vi "lvmcp_ctltype.vi"() -> ()   [LabVIEW 2026]
panel:
  out "error out":errorcluster
  out "data bytes":u8[](array[numeric])
  out "type string":i16[](array[numeric])
  in  "reference":refnum<vi>
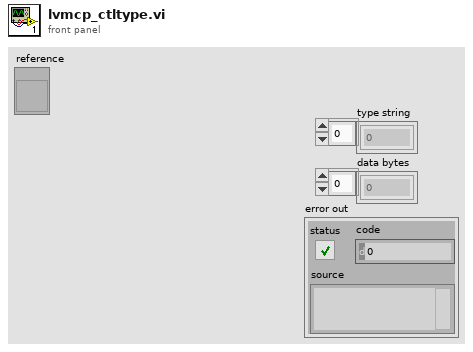
[diagram p1: front panel]
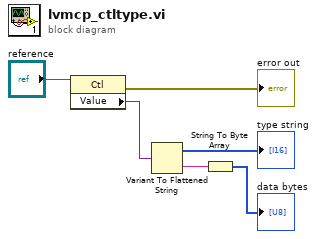
[diagram p0: block diagram]
diagram:
  n1 = property class="Ctl"(reference="reference") -> (error out=→"error out":errorcluster, "Value"=w5:variant)  [unwired: 1 in, 1 out]
  n2 = Variant To Flattened String(Variant=w5) -> (data string=w3:string, 1:→"type string":i16[])
  n3 = String To Byte Array(string=w3) -> (unsigned byte array=→"data bytes":u8[])
